vi "ControlList.vi"() -> (0 "Tab Control":cluster{"Control Path":string, "Data":variant}[](array[cluster]), 1 "BigCluster":cluster{"Control Path":string, "Data":variant}[](array[cluster]), 2 "Cluster":cluster{"Control Path":string, "Data":variant}[](array[cluster]), 3 "Basic":cluster{"Control Path":string, "Data":variant}[](array[cluster]), 4 "SubPanel":cluster{"Control Path":string, "Data":variant}[](array[cluster]), 6 "BasicArray":cluster{"Control Path":string, "Data":variant}[](array[cluster]))   [LabVIEW 2016, in "DronaTest.lvlib"]
uses:
  DronaTest.lvlib
  TestHelper/controls/Level2.ctl
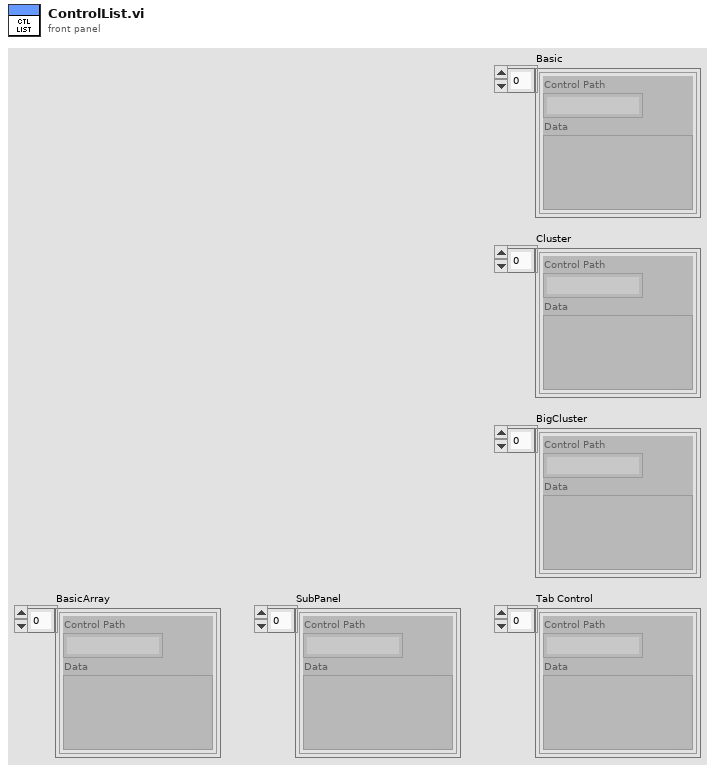
[diagram p1: front panel]
types:
  T1 = typedef "Level2.ctl" = cluster{"Numeric_cluster":dbl, "Boolean_cluster":bool, "target":string}
  T2 = cluster{"Numeric_cluster":dbl, "Boolean_cluster":bool, "String_cluster":string, "Level1":cluster{"Numeric_cluster":dbl, "Boolean_cluster":bool, "String_cluster":string, "Level2":T1}}
  T3 = cluster{"Numeric_cluster":dbl, "Boolean_cluster":bool, "String_cluster":string}
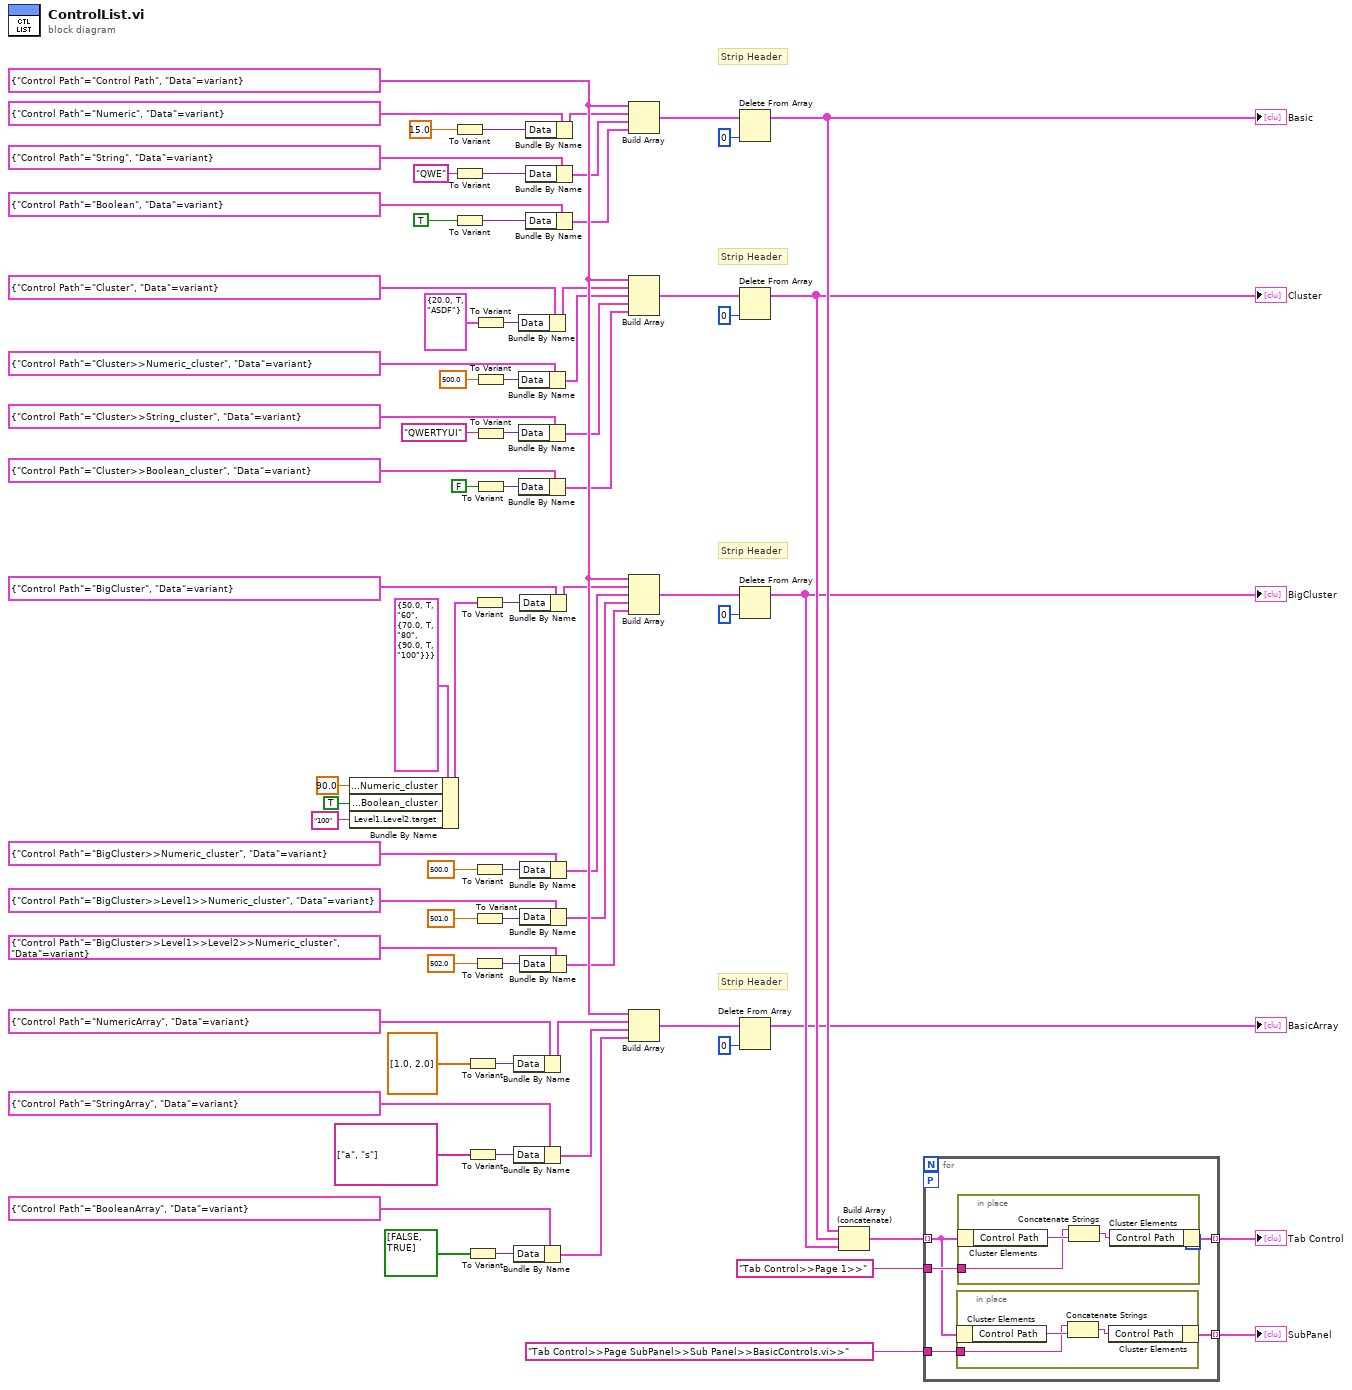
[diagram p0: block diagram]
diagram:
  w64 = cluster{"Control Path":string, "Data":variant} {"Control Path"="Control Path", "Data"=variant}
  # "Strip Header"
  # "Strip Header"
  # "Strip Header"
  # "Strip Header"
  n1 = Bundle By Name(cluster=T2 {"Numeric_cluster"=50.0, "Boolean_cluster"=TRUE, "String_cluster"="60", "Level1"={"Numeric_cluster"=70.0, "Boolean_cluster"=TRUE, "String_cluster"="80", "Level2"={"Numeric_cluster"=90.0, "Boolean_cluster"=TRUE, "target"="100"}}} ("BigCluster"), "Level1.Level2.Numeric_cluster"=90.0 ("Numeric_cluster"), "Level1.Level2.Boolean_cluster"=TRUE ("Boolean_cluster"), "Level1.Level2.target"="100" ("target")) -> (w20:T2)
  n2 = To Variant(anything=15.0 ("Data")) -> (Variant=w51:variant)
  n3 = To Variant(anything="QWE" ("Data")) -> (Variant=w50:variant)
  n4 = To Variant(anything=TRUE) -> (Variant=w49:variant)
  n5 = To Variant(anything=dbl[] [1.0, 2.0] ("Data")) -> (Variant=w3:variant)
  n6 = To Variant(anything=string[] ["a", "s"] ("Data")) -> (Variant=w2:variant)
  n7 = To Variant(anything=bool[] [FALSE, TRUE]) -> (Variant=w1:variant)
  n8 = To Variant(anything=w20) -> (Variant=w16:variant)
  n9 = To Variant(anything=500.0 ("Data")) -> (Variant=w15:variant)
  n10 = To Variant(anything=501.0 ("Data")) -> (Variant=w14:variant)
  n11 = To Variant(anything=502.0 ("Data")) -> (Variant=w13:variant)
  n12 = To Variant(anything=T3 {"Numeric_cluster"=20.0, "Boolean_cluster"=TRUE, "String_cluster"="ASDF"} ("Data")) -> (Variant=w36:variant)
  n13 = To Variant(anything=500.0 ("Data")) -> (Variant=w35:variant)
  n14 = To Variant(anything="QWERTYUI" ("Data")) -> (Variant=w34:variant)
  n15 = To Variant(anything=FALSE) -> (Variant=w33:variant)
  n16 = Bundle By Name(cluster=cluster{"Control Path":string, "Data":variant} {"Control Path"="NumericArray", "Data"=variant}, "Data"=w3) -> (w9:cluster{"Control Path":string, "Data":variant})
  n17 = Bundle By Name(cluster=cluster{"Control Path":string, "Data":variant} {"Control Path"="StringArray", "Data"=variant}, "Data"=w2) -> (w8:cluster{"Control Path":string, "Data":variant})
  n18 = Bundle By Name(cluster=cluster{"Control Path":string, "Data":variant} {"Control Path"="BooleanArray", "Data"=variant}, "Data"=w1) -> (w7:cluster{"Control Path":string, "Data":variant})
  n19 = Bundle By Name(cluster=cluster{"Control Path":string, "Data":variant} {"Control Path"="Cluster", "Data"=variant}, "Data"=w36) -> (w44:cluster{"Control Path":string, "Data":variant})
  n20 = Bundle By Name(cluster=cluster{"Control Path":string, "Data":variant} {"Control Path"="Cluster>>Numeric_cluster", "Data"=variant}, "Data"=w35) -> (w43:cluster{"Control Path":string, "Data":variant})
  n21 = Bundle By Name(cluster=cluster{"Control Path":string, "Data":variant} {"Control Path"="Cluster>>String_cluster", "Data"=variant}, "Data"=w34) -> (w42:cluster{"Control Path":string, "Data":variant})
  n22 = Bundle By Name(cluster=cluster{"Control Path":string, "Data":variant} {"Control Path"="Cluster>>Boolean_cluster", "Data"=variant}, "Data"=w33) -> (w41:cluster{"Control Path":string, "Data":variant})
  n23 = Bundle By Name(cluster=cluster{"Control Path":string, "Data":variant} {"Control Path"="BigCluster", "Data"=variant}, "Data"=w16) -> (w24:cluster{"Control Path":string, "Data":variant})
  n24 = Bundle By Name(cluster=cluster{"Control Path":string, "Data":variant} {"Control Path"="BigCluster>>Numeric_cluster", "Data"=variant}, "Data"=w15) -> (w23:cluster{"Control Path":string, "Data":variant})
  n25 = Bundle By Name(cluster=cluster{"Control Path":string, "Data":variant} {"Control Path"="BigCluster>>Level1>>Numeric_cluster", "Data"=variant}, "Data"=w14) -> (w22:cluster{"Control Path":string, "Data":variant})
  n26 = Bundle By Name(cluster=cluster{"Control Path":string, "Data":variant} {"Control Path"="BigCluster>>Level1>>Level2>>Numeric_cluster", "Data"=variant}, "Data"=w13) -> (w21:cluster{"Control Path":string, "Data":variant})
  n27 = Bundle By Name(cluster=cluster{"Control Path":string, "Data":variant} {"Control Path"="Numeric", "Data"=variant}, "Data"=w51) -> (w57:cluster{"Control Path":string, "Data":variant})
  n28 = Bundle By Name(cluster=cluster{"Control Path":string, "Data":variant} {"Control Path"="String", "Data"=variant}, "Data"=w50) -> (w56:cluster{"Control Path":string, "Data":variant})
  n29 = Bundle By Name(cluster=cluster{"Control Path":string, "Data":variant} {"Control Path"="Boolean", "Data"=variant}, "Data"=w49) -> (w55:cluster{"Control Path":string, "Data":variant})
  n30 = Build Array(w64, w57, w56, w55) -> (w77:cluster{"Control Path":string, "Data":variant}[])
  n31 = Build Array(w64, w44, w43, w42, w41) -> (w75:cluster{"Control Path":string, "Data":variant}[])
  n32 = Build Array(w64, w24, w23, w22, w21) -> (w74:cluster{"Control Path":string, "Data":variant}[])
  n33 = Build Array(w64, w9, w8, w7) -> (w66:cluster{"Control Path":string, "Data":variant}[])
  n34 = Delete From Array(array=w77, index=0) -> (array with subset deleted=w72:cluster{"Control Path":string, "Data":variant}[])  [unwired: 1 in, 1 out]
  "Basic" <- w72
  n35 = Delete From Array(array=w75, index=0) -> (array with subset deleted=w71:cluster{"Control Path":string, "Data":variant}[])  [unwired: 1 in, 1 out]
  "Cluster" <- w71
  n36 = Delete From Array(array=w74, index=0) -> (array with subset deleted=w70:cluster{"Control Path":string, "Data":variant}[])  [unwired: 1 in, 1 out]
  "BigCluster" <- w70
  n37 = Delete From Array(array=w66, index=0) -> (array with subset deleted=→"BasicArray":cluster{"Control Path":string, "Data":variant}[])  [unwired: 1 in, 1 out]
  n38 = Build Array (concatenate)(w72, w71, w70) -> (w67:cluster{"Control Path":string, "Data":variant}[])
  n39 = for {
    tunnel: w67 -> [w81] mode=indexing
    tunnel: [w83] -> w68 mode=indexing
    tunnel: "Tab Control>>Page 1>>" ("Control Path") -> [w82]
    tunnel: "Tab Control>>Page SubPanel>>Sub Panel>>BasicControls.vi>>" ("Control Path") -> [w80]
    tunnel: [w79] -> w61 mode=indexing
    workers-P: _ -> [_]
    n40 = in-place {
      in-place-border: w80 -> [w84]
      n41 = in-place-cluster #1(w81) -> ("Control Path"=w85:string)
      n42 = Concatenate Strings(w84, w85) -> (w86:string)
      n43 = in-place-cluster #1("Control Path"=w86) -> (w79:cluster{"Control Path":string, "Data":variant})
    }
    n44 = in-place {
      in-place-border: w82 -> [w87]
      n45 = in-place-cluster #2(w81) -> ("Control Path"=w88:string)
      n46 = Concatenate Strings(w87, w88) -> (w89:string)
      n47 = in-place-cluster #2("Control Path"=w89) -> (w83:cluster{"Control Path":string, "Data":variant})
    }
  }
  "Tab Control" <- w68
  "SubPanel" <- w61
